vi "Fetch Robot Changes.vi"() -> ()   [LabVIEW 2023]
doc: "Tools >> Systemcore >> Fetch Robot Changes: gets the deploy the robot runs (for example edits made in the robot's IDE) into the project. When only the robot has changes the project is updated; when both have, the user replaces theirs with the robot's, merges or keeps theirs. Reloads the project when its files changed."
panel:
  out "Status":string
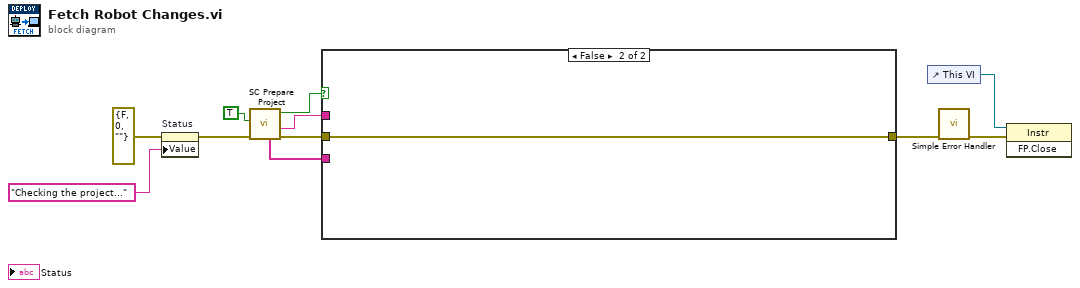
[diagram p0: block diagram]
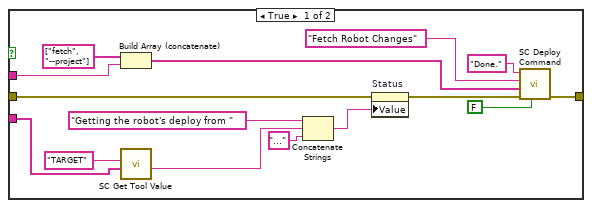
[diagram p2: hidden frame]
diagram:
  n1 = property on="Status" class="Str"(error in=errorcluster {"status"=FALSE, "code"=0, "source"=""}, "Value"="Checking the project...") -> (error out=w8:errorcluster)  [unwired: 1 in, 1 out]
  n2 = call "SC Prepare Project.vi"("error in (no error)"=w8, "save VIs?"=TRUE) -> ("error out"=w5:errorcluster, "project root"=w7:string, "ready?"=w4:bool, "tool lines"=w6:string[])  [unwired: 5 in, 1 out]
  n3 = case shown="False" w4 {
    tunnel: w7 -> [w18 _]
    tunnel: w6 -> [w26 _]
    tunnel: w5 -> [w21 w27]
    tunnel: [w12 w27] -> w3
    frame True {
      n4 = Build Array (concatenate)(string[] ["fetch", "--project"], w18) -> (w17:string[])
      n5 = call "SC Get Tool Value.vi"("tool lines"=w26, "key"="TARGET") -> ("value"=w23:string)  [unwired: 8 in, 1 out]
      n6 = Concatenate Strings("Getting the robot's deploy from ", w23, "...") -> (w20:string)
      n7 = property on="Status" class="Str"(error in=w21, "Value"=w20) -> (error out=w13:errorcluster)  [unwired: 1 in, 1 out]
      n8 = call "SC Deploy Command.vi"("deploying?"=FALSE, "error in (no error)"=w13, "arguments"=w17, "title"="Fetch Robot Changes", "OK message"="Done.") -> ("error out"=w12:errorcluster)  [unwired: 5 in, 1 out]
    }
    frame False {
    }
  }
  n9 = control-ref of="This VI"() -> (w2:refnum<vi>)
  n10 = call <vilib>:"Simple Error Handler.vi"("error in (no error)"=w3) -> ("error out"=w1:errorcluster)  [unwired: 4 in, 4 out]
  n11 = invoke class="Instr" method="FP.Close"(reference=w2, error in=w1) -> ()  [unwired: 1 in, 3 out]
